vi "GpuMat ConvertTo.vi"(5 "Beta":dbl, 6 "rType":T1, 7 "Alpha":dbl=1.0, 8 "error in (no error)":errorcluster, 9 "Stream in":refnum<class "Stream.lvclass">, 10 "Dst in":refnum<class "GpuMat.lvclass">, 11 "Src in":refnum<class "GpuMat.lvclass">) -> (0 "error out":errorcluster, 1 "Stream out":refnum<class "Stream.lvclass">, 3 "Dst out":refnum<class "GpuMat.lvclass">)   [LabVIEW 2020, in "OpenLvVision_OpenCv.lvlib" / "Cuda.lvlib" / "GpuMat.lvclass"]
doc: "Converts GpuMat to another datatype with scaling.\nThe underlying mathematical formula applied is: `dst(I) = saturate_cast<rtype>(src(I) * alpha + beta)`."
uses:
  GpuMat.lvclass
  OpenLvVision_OpenCv.lvlib
  <vilib>/Utility/error.llb/Error Cluster From Error Code.vi
  <vilib>/ErrorRing/Error Ring.xnode
  _LvHelpers/EdvrObject/EdvrObject.lvclass
  Dlls/OlvOpenCvWrapper.dll
  Stream/Stream.lvclass
  C:/Users/lukas/Documents/OpenLvVision_OpenCv/SourceCode/LabView/OpenLvVision_OpenCv/_LvHelpers/EdvrObject/EdvrObject.lvclass
  TypeDef/rType.ctl
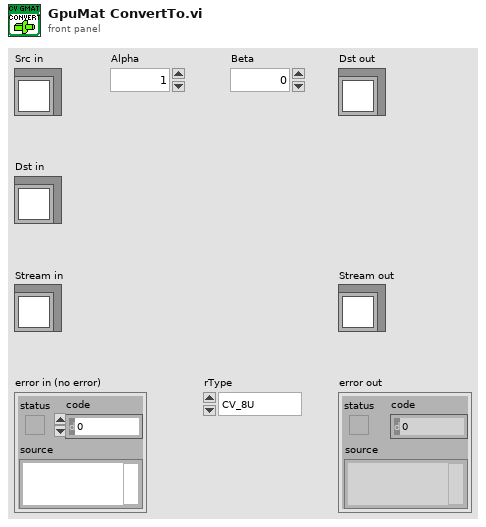
[diagram p1: front panel]
types:
  T1 = typedef "OpenLvVision_OpenCv.lvlib/rType.ctl" = enum32{"CV_8U", "CV_8S", "CV_16U", "CV_16S", "CV_32S", "CV_32F", "CV_64F"}
  T2 = typedef "OpenLvVision_OpenCv.lvlib/EdvrObject.lvclass/Edvr.ctl" = refnum<data-value>
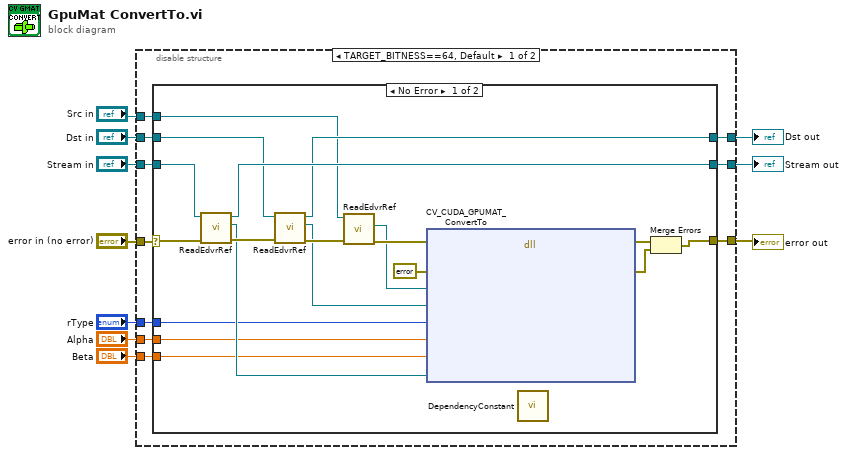
[diagram p0: block diagram]
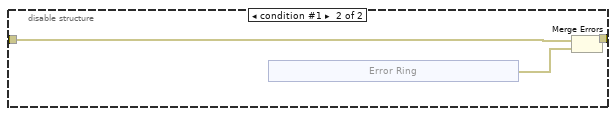
[diagram p3: hidden frame]
diagram:
  n1 = disable-structure shown="TARGET_BITNESS==64, Default" {
    disable-tunnel: "error in (no error)" -> [w20 w44]
    disable-tunnel: [w19 w45] -> w10
    disable-tunnel: "Src in" -> [w18 _]
    disable-tunnel: [w17 _] -> w4
    disable-tunnel: "Stream in" -> [w16 _]
    disable-tunnel: [w15 _] -> w6
    disable-tunnel: "Dst in" -> [w14 _]
    disable-tunnel: "rType" -> [w13 _]
    disable-tunnel: "Alpha" -> [w12 _]
    disable-tunnel: "Beta" -> [w11 _]
    frame condition #0 (active) {
      n2 = case shown="No Error" w20 {
        selector: w20 -> [w29 w42]
        tunnel: [w34 w42] -> w19
        tunnel: w18 -> [w21 _]
        tunnel: [w25 w40] -> w17
        tunnel: w16 -> [w27 w41]
        tunnel: [w28 w41] -> w15
        tunnel: w14 -> [w26 w40]
        tunnel: w13 -> [w24 _]
        tunnel: w12 -> [w23 _]
        tunnel: w11 -> [w22 _]
        frame No Error {
          n3 = call "ReadEdvrRef.vi"("error in (no error)"=w29, "EdvrObject in"=w27) -> ("error out"=w31:errorcluster, "Edvr"=w30:T2, "EdvrObject out"=w28:refnum<class "Stream.lvclass">)  [unwired: 7 in]
          n4 = call "ReadEdvrRef.vi"("error in (no error)"=w31, "EdvrObject in"=w26) -> ("error out"=w33:errorcluster, "Edvr"=w32:T2, "EdvrObject out"=w25:refnum<class "GpuMat.lvclass">)  [unwired: 7 in]
          n5 = call "ReadEdvrRef.vi"("error in (no error)"=w33, "EdvrObject in"=w21) -> ("error out"=w36:errorcluster, "Edvr"=w35:T2)  [unwired: 7 in, 1 out]
          n6 = dll-call lib="C:/Users/lukas/Documents/OpenLvVision_OpenCv/SourceCode/LabView/OpenLvVision_OpenCv/Dlls/OlvOpenCvWrapper.dll" fn="CV_CUDA_GPUMAT_ConvertTo"(error in=w36, "Error"=errorcluster {"status"=FALSE, "code"=0, "source"=""} ("error out"), "srcRef"=w35, "dstRef"=w32, "rtype"=w24, "alpha"=w23, "beta"=w22, "streamRef"=w30) -> (error out=w39:errorcluster, "Error"=w38:errorcluster)  [unwired: 9 in, 1 out]
          n7 = call "DependencyConstant.vi"() -> ()  [unwired: 12 in]
          n8 = Merge Errors(w39, w38) -> (w34:errorcluster)
        }
        frame Error {
        }
      }
    }
    frame condition #1 {
      n9 = xnode "Error Ring"() -> ("error out"=w43:errorcluster)
      n10 = Merge Errors(w44, w43) -> (w45:errorcluster)
    }
  }
  "error out" <- w10
  "Stream out" <- w6
  "Dst out" <- w4
